vi "_LabeledRectangleDrawText.vi"(4 "Text":string, 5 "TextColor":u32(colorbox)=16711680, 6 "TextSettings":T1, 7 "GroupName":string, 8 "error in":errorcluster, 9 "TextHeigth":i32, 10 "BoundingBox":T2, 11 "Image Reference In":T4) -> (0 "error out":errorcluster, 3 "Image Reference Out":T4)   [LabVIEW 2020, in "OpenLvVision_Overlays.lvlib"]
uses:
  OpenLvVision_Overlays.lvlib
  <vilib>/OpenLvVision/OpenLvVision_Image/Management/TypeDef/OLV Image.ctl
  TypeDefs/RotatedRectangle.ctl
  TypeDefs/PointI32.ctl
  TypeDefs/TextSettings.ctl
  TypeDefs/Line.ctl
  <vilib>/OpenLvVision/OpenLvVision_Image/Management/OLV Management.lvlib
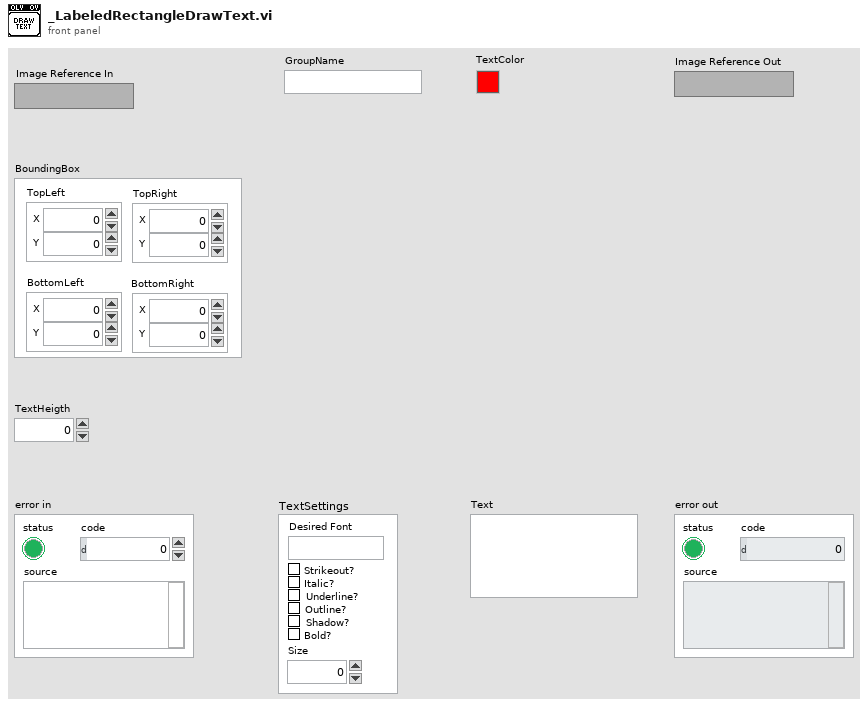
[diagram p1: front panel]
types:
  T1 = typedef "OpenLvVision_Overlays.lvlib/TextSettings.ctl" = cluster{"Desired Font":string, "Strikeout?":bool, "Italic?":bool, "Underline?":bool, "Outline?":bool, "Shadow?":bool, "Bold?":bool, "Size":i32}
  T2 = typedef "OpenLvVision_Overlays.lvlib/RotatedRectangle.ctl" = cluster{"TopLeft":T3, "TopRight":T3, "BottomRight":T3, "BottomLeft":T3}
  T3 = typedef "OpenLvVision_Overlays.lvlib/PointI32.ctl" = cluster{"X":i32, "Y":i32}
  T4 = typedef "OLV OpenLvVision_Image.lvlib/OLV Management.lvlib/OLV Image.ctl" = refnum<image>
  T5 = cluster{"Desired Font (Application)":enum16{"User-specified Font", "Application Font", "System Font", "Dialog Font"}, "[User-specified Font]":cluster{"Font Name":string, "Size":i16, "Strikeout?":bool, "Italic?":bool, "Underline?":bool, "Outline?":bool, "Shadow?":bool, "Bold?":bool, "Rotation Angle":dbl}, "Horizontal Alignment":i16, "Vertical Alignment":i16}
  T6 = typedef "OpenLvVision_Overlays.lvlib/Line.ctl" = cluster{"StartPoint":T3, "EndPoint":T3}
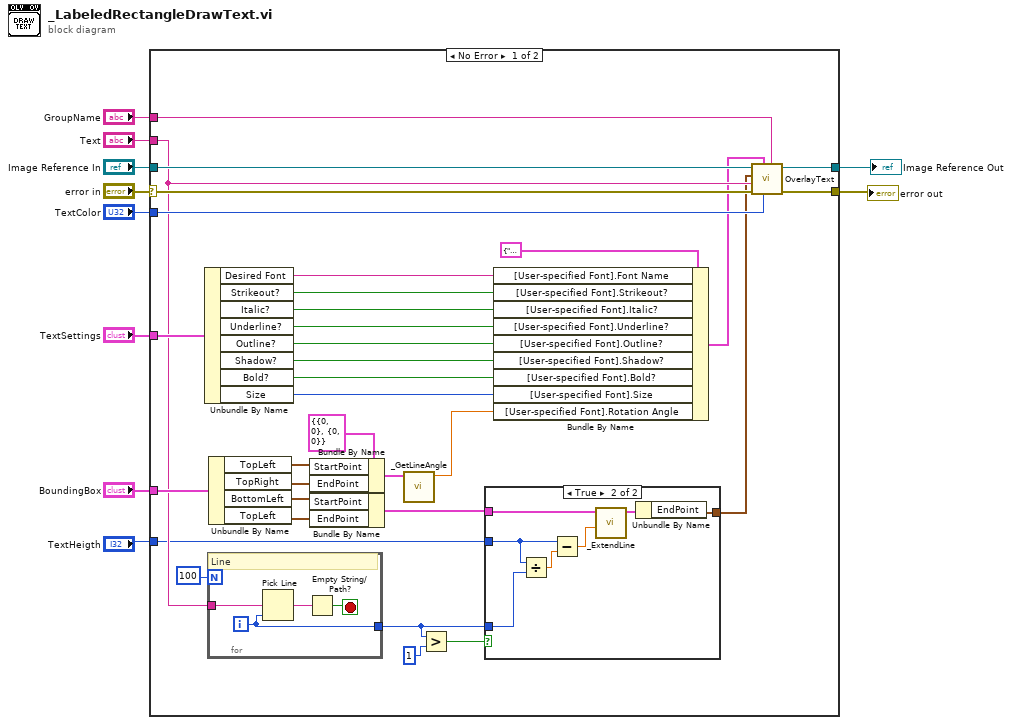
[diagram p0: block diagram]
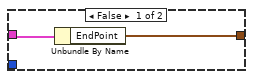
[diagram p2: hidden frame]
diagram:
  n1 = case shown="No Error" "error in" {
    selector: "error in" -> [w40 w57]
    tunnel: [w43 w57] -> w9
    tunnel: "Image Reference In" -> [w41 w58]
    tunnel: [w42 w58] -> w8
    tunnel: "GroupName" -> [w39 _]
    tunnel: "TextColor" -> [w38 _]
    tunnel: "Text" -> [w19 _]
    tunnel: "TextSettings" -> [w36 _]
    tunnel: "BoundingBox" -> [w28 _]
    tunnel: "TextHeigth" -> [w13 _]
    frame No Error {
      w24 = T6 {"StartPoint"={"X"=0, "Y"=0}, "EndPoint"={"X"=0, "Y"=0}} ("Line")
      n2 = Unbundle By Name(w36) -> ("Desired Font"=w35:string, "Strikeout?"=w34:bool, "Italic?"=w33:bool, "Underline?"=w32:bool, "Outline?"=w31:bool, "Shadow?"=w30:bool, "Bold?"=w29:bool, "Size"=w20:i32)
      n3 = for {
        N: 100 -> [_]
        tunnel: w19 -> [w47]
        tunnel: [w44] -> w16
        i -> [w44]
        stop <- w45 stop-if-true
        # "Line"
        n4 = Pick Line(multi-line string=w47, line index=w44) -> (output string=w46:string)  [unwired: 1 in]
        n5 = Empty String/Path?(string/path=w46) -> (empty?=w45:bool)
      }
      n6 = Unbundle By Name(w28) -> ("TopLeft"=w27:T3, "TopRight"=w26:T3, "BottomLeft"=w22:T3, "TopLeft"=w21:T3)
      n7 = Bundle By Name(cluster=w24, "StartPoint"=w27, "EndPoint"=w26) -> (w25:T6)
      n8 = Bundle By Name(cluster=w24, "StartPoint"=w22, "EndPoint"=w21) -> (w23:T6)
      n9 = call "_GetLineAngle.vi"("Line"=w25) -> ("Angle"=w14:dbl)  [unwired: 10 in]
      n10 = Greater?(x=w16, y=1) -> (0:w17:bool)
      n11 = case shown="True" w17 {
        tunnel: w23 -> [w49 w56]
        tunnel: [w48 w54] -> w12
        tunnel: w16 -> [_ w52]
        tunnel: w13 -> [_ w50]
        frame False {
          n12 = Unbundle By Name(w49) -> ("EndPoint"=w48:T3)
        }
        frame True {
          n13 = Divide(x=w50, y=w52) -> (x/y=w51:dbl)
          n14 = Subtract(x=w50, y=w51) -> (x-y=w53:dbl)
          n15 = call "_ExtendLine.vi"("ExtendEnd"=w53, "Line"=w56) -> ("Line"=w55:T6)  [unwired: 9 in]
          n16 = Unbundle By Name(w55) -> ("EndPoint"=w54:T3)
        }
      }
      n17 = Bundle By Name(cluster=T5 {"Desired Font (Application)"=enum."User-specified Font", "[User-specified Font]"={"Font Name"="", "Size"=12, "Strikeout?"=FALSE, "Italic?"=FALSE, "Underline?"=FALSE, "Outline?"=FALSE, "Shadow?"=FALSE, "Bold?"=FALSE, "Rotation Angle"=0.0}, "Horizontal Alignment"=0, "Vertical Alignment"=0} ("Font, Size & Style"), "[User-specified Font].Font Name"=w35, "[User-specified Font].Strikeout?"=w34, "[User-specified Font].Italic?"=w33, "[User-specified Font].Underline?"=w32, "[User-specified Font].Outline?"=w31, "[User-specified Font].Shadow?"=w30, "[User-specified Font].Bold?"=w29, "[User-specified Font].Size"=w20, "[User-specified Font].Rotation Angle"=w14) -> (w11:T5)
      n18 = call "OverlayText.vi"("GroupName"=w39, "Text Color (black)"=w38, "Font, Size & Style"=w11, "error in"=w40, "Text"=w19, "Origin"=w12, "Image Reference In"=w41) -> ("error out"=w43:errorcluster, "Image Reference Out"=w42:T4)  [unwired: 3 in]
    }
    frame Error {
    }
  }
  "error out" <- w9
  "Image Reference Out" <- w8
